vi "值比较.vi"(5 "上限":dbl, 7 "下限":dbl, 9 "x":dbl, 10 "s":bool=TRUE) -> (1 "颜色盒":u32(colorbox)=16711680, 2 "值":string, 3 "Pass(T)/Fail(F)":bool, 4 "结果":enum16{"Failed", "Passed", "Disabled"}(ring))   [LabVIEW 2025]
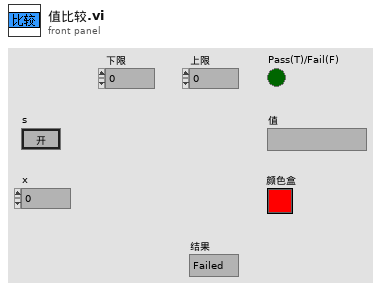
[diagram p1: front panel]
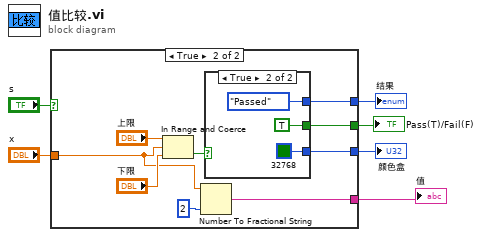
[diagram p0: block diagram]
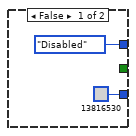
[diagram p2: hidden frame]
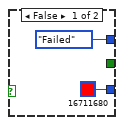
[diagram p3: hidden frame]
diagram:
  n1 = case shown="True" "s" {
    tunnel: [u32 13816530 ("颜色盒") w13] -> w3
    tunnel: [enum16{"Failed", "Passed", "Disabled"}."Disabled" w14] -> w2
    tunnel: "x" -> [_ w11]
    tunnel: [_ w10] -> w4
    tunnel: [_ w9] -> w1
    frame False {
    }
    frame True {
      n2 = In Range and Coerce(upper limit="上限", x=w11, lower limit="下限") -> (In Range?=w17:bool)  [unwired: 1 out]
      n3 = Number To Fractional String(number=w11, precision (6)=i16 2 ("精度(6)")) -> (F-format string=w10:string)  [unwired: 2 in]
      n4 = case shown="True" w17 {
        tunnel: [u32 16711680 ("颜色盒") u32 32768 ("颜色盒")] -> w13
        tunnel: [enum16{"Failed", "Passed", "Disabled"}."Failed" enum16{"Failed", "Passed", "Disabled"}."Passed"] -> w14
        tunnel: [_ TRUE] -> w9
        frame False {
        }
        frame True {
        }
      }
    }
  }
  "颜色盒" <- w3
  "值" <- w4
  "结果" <- w2
  "Pass(T)/Fail(F)" <- w1
